vi "three phase power monitor.vi"() -> ()   [LabVIEW 2026]
panel:
  in  "stop":bool
  out "Waveform Chart":cluster{dbl, dbl, dbl}(graph)
  out "Total Power Factor":dbl
  out "Phase R Voltage":dbl
  out "Phase B Voltage":dbl
  out "Phase Y Voltage":dbl
  out "Reactive Power":dbl
  out "Active Power":dbl
  out "Apparent Power":dbl
  out "Line Voltage":dbl
  in  "Power Factor":dbl
  in  "Frequency":dbl
  in  "Phase Current":dbl
  in  "Phase Voltage":dbl
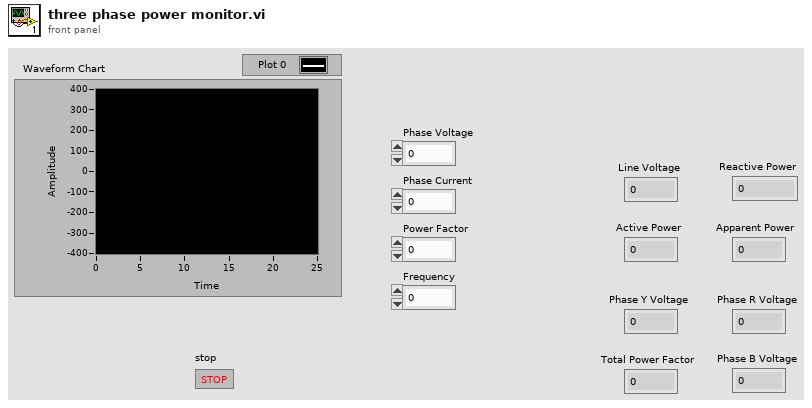
[diagram p1: front panel]
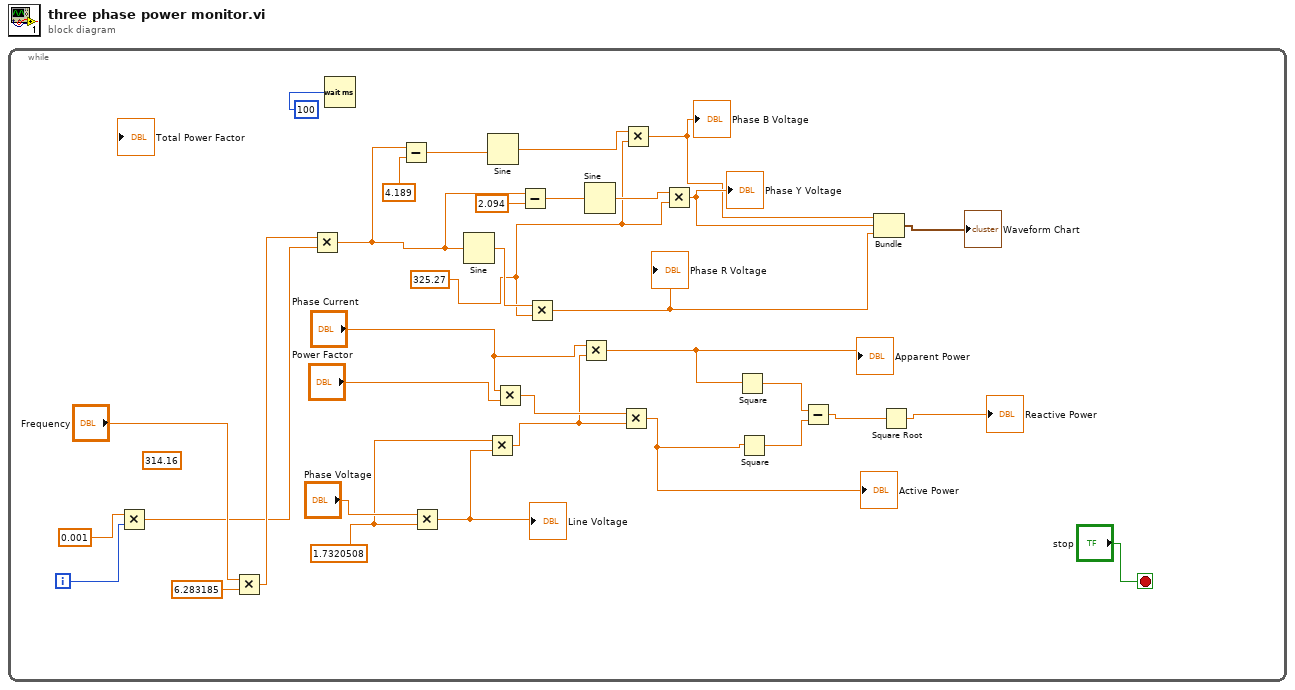
[diagram p0: block diagram]
diagram:
  n1 = while {
    i -> [w18]
    stop <- "stop" stop-if-true
    w9 = 325.27 ("y")
    (unwired) 314.16 ("y")
    w32 = 1.7320508
    n2 = Multiply(x=0.001, y=w18) -> (x*y=w1:dbl)
    n3 = Multiply(x="Frequency", y=6.283185) -> (x*y=w2:dbl)
    n4 = Multiply(x=w2, y=w1) -> (x*y=w14:dbl)
    n5 = Wait (ms)(milliseconds to wait=u32 100) -> ()  [unwired: 1 out]
    n6 = Subtract(x=w14, y=4.189) -> (x-y=w12:dbl)
    n7 = Multiply(x="Phase Voltage", y=w32) -> (x*y=w33:dbl)
    "Line Voltage" <- w33
    n8 = Sine(x=w14) -> (sin(x)=w17:dbl)
    n9 = Multiply(x=w32, y=w33) -> (x*y=w28:dbl)
    n10 = Sine(x=w12) -> (sin(x)=w10:dbl)
    n11 = Multiply(x="Phase Current", y="Power Factor") -> (x*y=w30:dbl)
    n12 = Subtract(x=w14, y=2.094) -> (x-y=w15:dbl)
    n13 = Multiply(x=w17, y=w9) -> (x*y=w7:dbl)
    "Phase R Voltage" <- w7
    n14 = Multiply(x="Phase Current", y=w28) -> (x*y=w27:dbl)
    "Apparent Power" <- w27
    n15 = Sine(x=w15) -> (sin(x)=w11:dbl)
    n16 = Multiply(x=w30, y=w28) -> (x*y=w24:dbl)
    "Active Power" <- w24
    n17 = Multiply(x=w10, y=w9) -> (x*y=w5:dbl)
    "Phase B Voltage" <- w5
    n18 = Multiply(x=w11, y=w9) -> (x*y=w6:dbl)
    "Phase Y Voltage" <- w6
    n19 = Square(x=w27) -> (x^2=w26:dbl)
    n20 = Square(x=w24) -> (x^2=w25:dbl)
    n21 = Subtract(x=w26, y=w25) -> (x-y=w23:dbl)
    n22 = Bundle(w5, w6, w7) -> (→"Waveform Chart":cluster{dbl, dbl, dbl})  [unwired: 1 in]
    n23 = Square Root(x=w23) -> (sqrt(x)=→"Reactive Power":dbl)
  }
